vi "Read.vi"(8 "error in (no error)":errorcluster, 9 "timeout ms":i32, 10 "frames in":T1 {"flags" format="%.0x"; "id" format="%.0x"}, 11 "channel in":refnum<class "CANsub_DirectChannel.lvclass">) -> (0 "error out":errorcluster, 2 "frames out":T1 {"flags" format="%.0x"; "id" format="%.0x"}, 3 "channel out":refnum<class "CANsub_DirectChannel.lvclass">)   [LabVIEW 2021, in "CANsub_API.lvlib" / "CANsub_DirectChannel.lvclass"]
doc: "Direct: Poll-mode read; calls Read_Poll in place on the object’s TLS connection, decoder state, pending bytes and status. Loop-safe: no allocation, bounded time."
uses:
  CANsub_DirectChannel.lvclass
  CANsub_DirectChannel.lvclass/CANsub_DirectChannel.ctl
  CANsub_API.lvlib
  Typedefs/CANsub_Frames.ctl
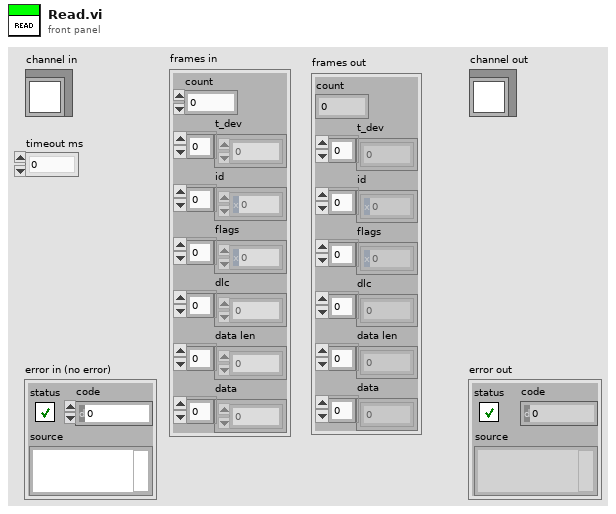
[diagram p1: front panel]
types:
  T1 = typedef "CANsub_API.lvlib/CANsub_Frames.ctl" = cluster{"count":i32, "t_dev":dbl[], "id":u32[], "flags":u16[], "dlc":u8[], "data len":u8[], "data":u8[]}
  T2 = typedef "CANsub_C.lvlib/C_RX_State.ctl" = cluster{"ws":u8[], "hdlc":u8[], "ping":u8[]}
  T3 = typedef "CANsub_API.lvlib/CANsub_Status.ctl" = cluster{"state":T4, "frames read":u32, "frames written":u32, "crc errors":u32, "decode errors":i32, "pings":u32, "FIFO overflows":u32, "reopens":u32, "nodelay":i32, "api version":string, "lib version":u32, "bit timing":T5, "last error":errorcluster}
  T4 = typedef "CANsub_API.lvlib/CANsub_State.ctl" = enum16{"Closed", "Open", "Lost"}
  T5 = typedef "CANsub_Common.lvlib/Bit_Timing.ctl" = cluster{"brp":u16, "seg1":u16, "seg2":u16, "sjw":u16, "data brp":u16, "data seg1":u16, "data seg2":u16, "data sjw":u16}
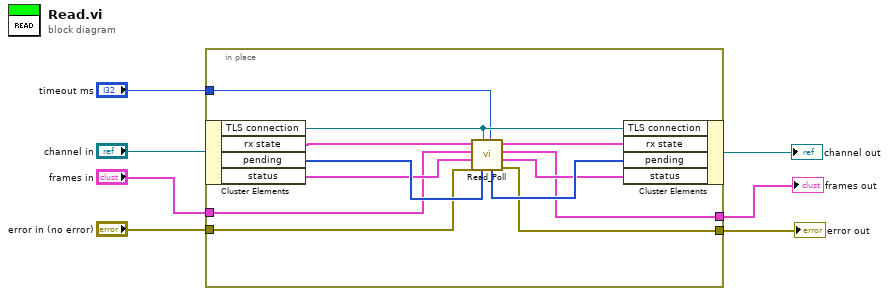
[diagram p0: block diagram]
diagram:
  n1 = in-place {
    in-place-border: "error in (no error)" -> [w12]
    in-place-border: [w11] -> w5
    in-place-border: "frames in" -> [w10]
    in-place-border: [w9] -> w2
    in-place-border: "timeout ms" -> [w8]
    n2 = in-place-cluster #1("channel in") -> ("TLS connection"=w19:refnum<k5>, "rx state"=w18:T2, "pending"=w16:u8[], "status"=w14:T3)
    n3 = call "Read_Poll.vi"("timeout ms"=w8, "pending in"=w16, "TLS connection"=w19, "error in (no error)"=w12, "status in"=w14, "frames in"=w10, "rx state in"=w18) -> ("error out"=w11:errorcluster, "status out"=w13:T3, "frames out"=w9:T1, "rx state out"=w17:T2, "pending out"=w15:u8[])
    n4 = in-place-cluster #1("TLS connection"=w19, "rx state"=w17, "pending"=w15, "status"=w13) -> (→"channel out":refnum<class "CANsub_DirectChannel.lvclass">)
  }
  "error out" <- w5
  "frames out" <- w2
